vi "laser_current_amplitude_sweep.vi"() -> ()   [LabVIEW 2025, in "tSNIP.lvlib"]
uses:
  tSNIP.lvlib
panel:
  in  "LASER":bool
  in  "Step":T1 {"Size"."Units" items=["mA"=0.001, "A"=1.0]; "Period"."Units" items=["s"=1, "min"=60]}
  in  "Final Current":cluster{"Amplitude":dbl, "Units":dbl} {"Units" items=["A"=1.0, "mA"=0.001]}
  in  "VISA resource name":refnum<visa-resource-name>
  in  "Start Current":cluster{"Amplitude":dbl, "Units":dbl}={"Amplitude"=0.0, "Units"=0.0010000000474974513} {"Units" items=["A"=1.0, "mA"=0.0010000000474974513]}
  in  "Exit":bool
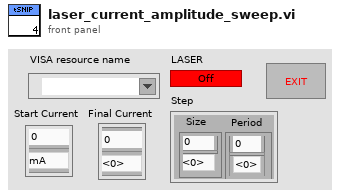
[diagram p1: front panel]
types:
  T1 = cluster{"Period":cluster{"Value":dbl, "Units":i8}, "Size":cluster{"Value":dbl, "Units":dbl}}
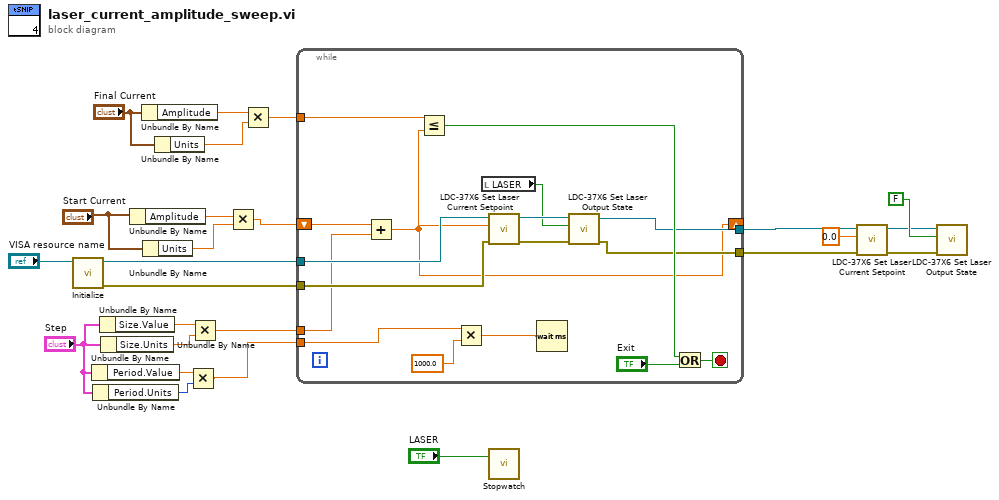
[diagram p0: block diagram]
diagram:
  n1 = call "Initialize.vi"("VISA resource name"="VISA resource name") -> ("error out"=w17:errorcluster, "VISA resource name out"=w18:refnum<visa-resource-name>)  [unwired: 9 in]
  n2 = Unbundle By Name("Step") -> ("Period.Value"=w8:dbl)
  n3 = Unbundle By Name("Step") -> ("Period.Units"=w7:i8)
  n4 = Unbundle By Name("Step") -> ("Size.Value"=w10:dbl)
  n5 = Unbundle By Name("Step") -> ("Size.Units"=w9:dbl)
  n6 = Unbundle By Name("Start Current") -> ("Amplitude"=w12:dbl)
  n7 = Unbundle By Name("Final Current") -> ("Amplitude"=w15:dbl)
  n8 = Unbundle By Name("Start Current") -> ("Units"=w13:dbl)
  n9 = Unbundle By Name("Final Current") -> ("Units"=w16:dbl)
  n10 = Multiply(x=w8, y=w7) -> (x*y=w4:dbl)
  n11 = Multiply(x=w10, y=w9) -> (x*y=w3:dbl)
  n12 = Multiply(x=w12, y=w13) -> (x*y=w2:dbl)
  n13 = Multiply(x=w15, y=w16) -> (x*y=w5:dbl)
  n14 = while {
    shift-right: [w27] -> _
    shift-left: w2 -> [w42]
    tunnel: [w36] -> w21
    tunnel: [w35] -> w20
    tunnel: w18 -> [w33]
    tunnel: w17 -> [w32]
    tunnel: w5 -> [w31]
    tunnel: w3 -> [w30]
    tunnel: w4 -> [w29]
    stop <- w28 stop-if-true
    n15 = Add(x=w42, y=w30) -> (x+y=w27:dbl)
    n16 = Less Or Equal?(x=w31, y=w27) -> (x <= y?=w37:bool)
    n17 = Multiply(x=w29, y=1000.0) -> (x*y=w34:dbl)
    n18 = local read "LASER"() -> (w26:bool)
    n19 = call <instrlib>:"LDC-37X6 Set Laser Current Setpoint.vi"("VISA resource name"=w33, "Laser Current Setpoint (A)"=w27, "error in"=w32) -> ("VISA resource name out"=w41:refnum<visa-resource-name>, "error out"=w40:errorcluster)  [unwired: 6 in]
    n20 = Wait (ms)(milliseconds to wait=w34) -> ()  [unwired: 1 out]
    n21 = call <instrlib>:"LDC-37X6 Set Laser Output State.vi"("error in"=w40, "Laser Output Enable"=w26, "VISA resource name"=w41) -> ("error out"=w35:errorcluster, "VISA resource name out"=w36:refnum<visa-resource-name>)  [unwired: 7 in]
    n22 = Or(x=w37, y="Exit") -> (x .or. y?=w28:bool)
  }
  n23 = call "Stopwatch.vi"("Start"="LASER") -> ()  [unwired: 18 in, 1 out]
  n24 = call <instrlib>:"LDC-37X6 Set Laser Current Setpoint.vi"("VISA resource name"=w21, "Laser Current Setpoint (A)"=0.0, "error in"=w20) -> ("VISA resource name out"=w22:refnum<visa-resource-name>, "error out"=w24:errorcluster)  [unwired: 6 in]
  n25 = call <instrlib>:"LDC-37X6 Set Laser Output State.vi"("error in"=w24, "Laser Output Enable"=FALSE, "VISA resource name"=w22) -> ()  [unwired: 7 in, 2 out]
